vi "Initialize Hardware.vi"(7 "RT config file":path, 8 "error in":errorcluster, 11 "device parameters":T5) -> (0 "error out":errorcluster, 3 "RT handles":T4, 5 "device information":T1)   [LabVIEW 2020, in "Ballard ARINC 429 Engine.lvlib" / "Custom Device.lvlib"]
uses:
  Custom Device.lvlib
  Shared/Device Parameters.ctl
  Shared/Initialization Method.ctl
  Hardware Handles.ctl
  Device Information.ctl
  Hardware Direction and Channels.ctl
  Shared/Direction Capability.ctl
  <instrlib>/BTICardLib/Private/Initialize By Card Number and Core Number.vi
  <instrlib>/BTICardLib/Private/Initialize By Slot Number and Core Number.vi
  <instrlib>/BTICardLib/Private/Initialize By Core Serial Number.vi
  <instrlib>/BTICardLib/Private/IO/Action-Status/Write External LED.vi
  <instrlib>/BTI429Lib/Private/Core/Action-Status/Start All Channels.vi
  <instrlib>/BTICardLib/Private/Configure All From XML.vi
  <instrlib>/BTICardLib/BTICardLV.lvlib
  <instrlib>/BTI429Lib/BTI429LV.lvlib
  <vilib>/NI VeriStand/Custom Device Tools/Custom Device Utility Library/Custom Device Utility Library.lvlib
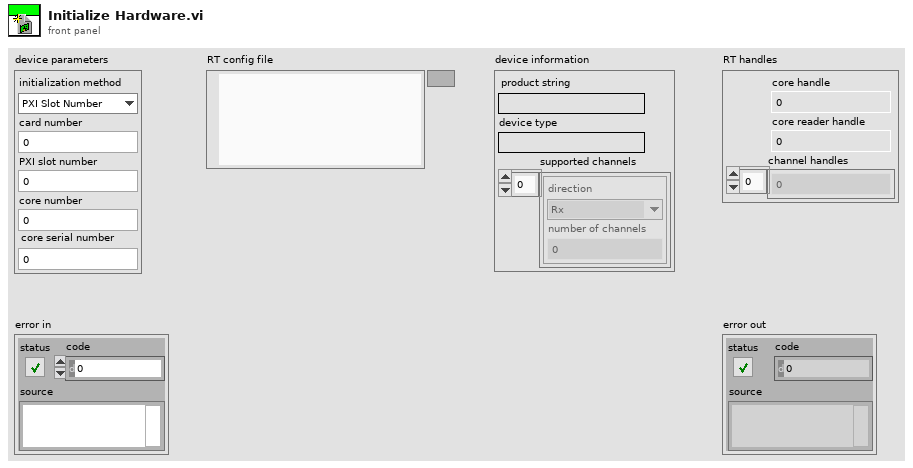
[diagram p1: front panel]
types:
  T1 = typedef "Ballard ARINC 429 Engine.lvlib/Custom Device.lvlib/Device Information.ctl" = cluster{"product string":string, "device type":string, "supported channels":T2[]}
  T2 = typedef "Ballard ARINC 429 Engine.lvlib/Custom Device.lvlib/Hardware Direction and Channels.ctl" = cluster{"direction":T3, "number of channels":u16}
  T3 = typedef "Direction Capability.ctl" = enum16{"Rx", "Tx", "Rx/Tx"}
  T4 = typedef "Ballard ARINC 429 Engine.lvlib/Custom Device.lvlib/Hardware Handles.ctl" = cluster{"core handle":u64, "core reader handle":u64, "channel handles":u64[]}
  T5 = typedef "Device Parameters.ctl" = cluster{"initialization method":T6, "card number":i32, "PXI slot number":i32, "core number":i32, "core serial number":i32}
  T6 = typedef "Initialization Method.ctl" = enum16{"PXI Slot Number", "Card Number", "Core Serial Number"}
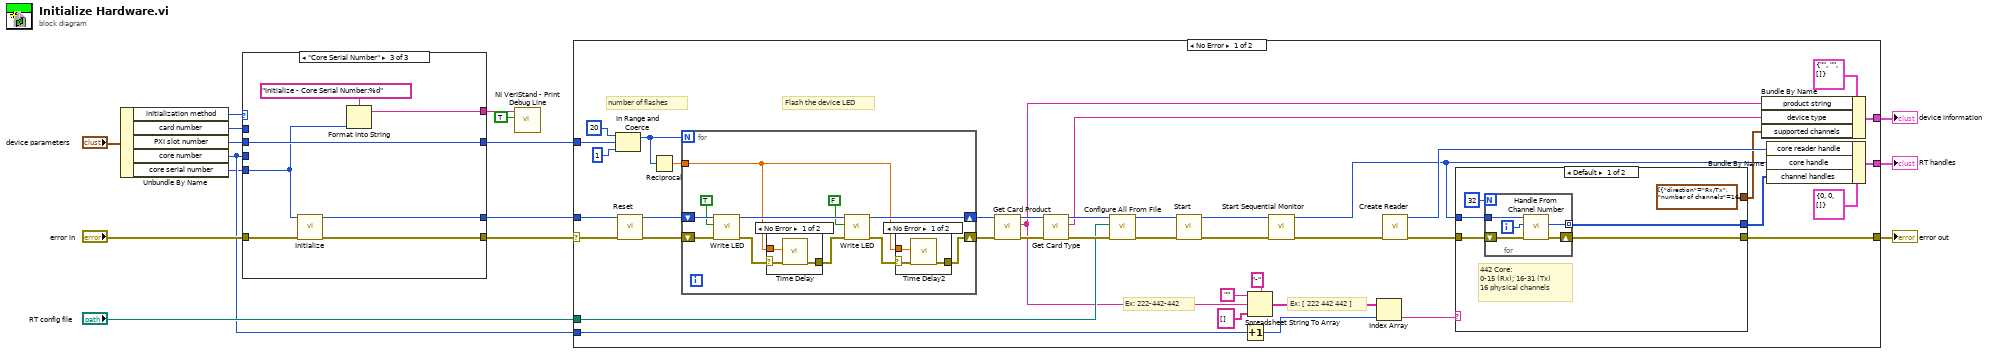
[diagram p0: block diagram]
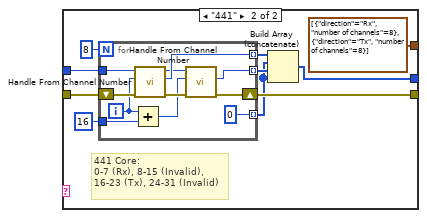
[diagram p2: hidden frame]
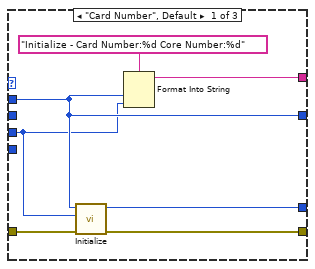
[diagram p6: hidden frame]
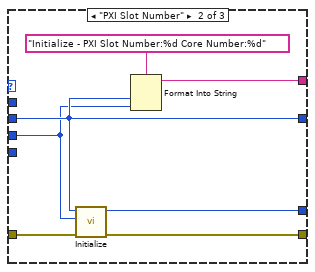
[diagram p7: hidden frame]
diagram:
  n1 = Unbundle By Name("device parameters") -> ("initialization method"=w16:T6, "card number"=w15:i32, "PXI slot number"=w14:i32, "core number"=w4:i32, "core serial number"=w3:i32)
  n2 = case shown="\"Core Serial Number\"" w16 {
    tunnel: [w23 w30 w37] -> w10
    tunnel: [w22 w29 w36] -> w12
    tunnel: w15 -> [w20 _ _]
    tunnel: "error in" -> [w21 w28 w35]
    tunnel: w14 -> [_ w27 w34]
    tunnel: w4 -> [w19 w26 _]
    tunnel: [w20 w27 w34] -> w9
    tunnel: w3 -> [_ _ w33]
    tunnel: [w17 w24 w31] -> w1
    frame "Card Number", Default {
      n3 = call-poly <instrlib>:"Initialize.vi"("error in (no error)"=w21, "core number"=w19, "card number"=w20) -> ("error out"=w22:errorcluster, "core handle out"=w23:u64)  [unwired: 7 in]
      n4 = Format Into String(format string="Initialize - Card Number:%d Core Number:%d", w20, w19) -> (resulting string=w17:string)  [unwired: 2 in, 1 out]
    }
    frame "PXI Slot Number" {
      n5 = call-poly <instrlib>:"Initialize.vi"("error in (no error)"=w28, "core number"=w26, "slot number"=w27) -> ("error out"=w29:errorcluster, "core handle out"=w30:u64)  [unwired: 7 in]
      n6 = Format Into String(format string="Initialize - PXI Slot Number:%d Core Number:%d", w27, w26) -> (resulting string=w24:string)  [unwired: 2 in, 1 out]
    }
    frame "Core Serial Number" {
      n7 = call-poly <instrlib>:"Initialize.vi"("error in (no error)"=w35, "core serial number"=w33) -> ("error out"=w36:errorcluster, "core handle out"=w37:u64)  [unwired: 8 in]
      n8 = Format Into String(format string="Initialize - Core Serial Number:%d", w33) -> (resulting string=w31:string)  [unwired: 2 in, 1 out]
    }
  }
  n9 = call <vilib>:"NI VeriStand - Print Debug Line.vi"("Add to log file? (F)"=TRUE, "Message"=w1) -> ()  [unwired: 9 in, 1 out]
  n10 = case shown="No Error" w12 {
    selector: w12 -> [w77 w128]
    tunnel: w10 -> [w76 _]
    tunnel: w9 -> [w73 _]
    tunnel: [w54 _] -> w8
    tunnel: [w52 _] -> w7
    tunnel: [w51 w128] -> w6
    tunnel: "RT config file" -> [w48 _]
    tunnel: w4 -> [w40 _]
    frame No Error {
      # "Ex: [ 222 442 442 ]"
      # "Ex: 222-442-442"
      # "number of flashes"
      # "Flash the device LED"
      n11 = In Range and Coerce(upper limit=20 ("x"), x=w73, lower limit=1) -> (coerced(x)=w69:i32)  [unwired: 1 out]
      n12 = call <instrlib>:"Reset.vi"("error in (no error)"=w77, "core handle in"=w76) -> ("error out"=w75:errorcluster, "core handle out"=w74:u64)  [unwired: 8 in]
      n13 = Reciprocal(x=w69) -> (1/x=w70:dbl)
      n14 = for {
        N: w69 -> [_]
        shift-right: [w118] -> w66
        shift-left: w74 -> [w117]
        shift-right: [w112] -> w65
        shift-left: w75 -> [w116]
        tunnel: w70 -> [w109]
        n15 = call-poly <instrlib>:"Write LED.vi"("error in (no error)"=w116, "LED state"=TRUE, "core handle in"=w117) -> ("error out"=w111:errorcluster, "core handle out"=w119:u64)  [unwired: 7 in]
        n16 = case shown="No Error" w111 {
          selector: w111 -> [w122 w123]
          tunnel: [w121 w123] -> w110
          tunnel: w109 -> [w120 _]
          frame No Error {
            n17 = call "Time Delay"("error in (no error)"=w122, "Delay Time (s)"=w120) -> ("error out"=w121:errorcluster)  [unwired: 9 in]
          }
          frame Error {
          }
        }
        n18 = call-poly <instrlib>:"Write LED.vi"("error in (no error)"=w110, "LED state"=FALSE, "core handle in"=w119) -> ("error out"=w113:errorcluster, "core handle out"=w118:u64)  [unwired: 7 in]
        n19 = case shown="No Error" w113 {
          selector: w113 -> [w126 w127]
          tunnel: [w125 w127] -> w112
          tunnel: w109 -> [w124 _]
          frame No Error {
            n20 = call "Time Delay2"("error in (no error)"=w126, "Delay Time (s)"=w124) -> ("error out"=w125:errorcluster)  [unwired: 9 in]
          }
          frame Error {
          }
        }
      }
      n21 = call <instrlib>:"Get Card Product.vi"("error in (no error)"=w65, "core handle in"=w66) -> ("error out"=w67:errorcluster, "product string out"=w42:string, "core handle out"=w68:u64)  [unwired: 7 in]
      n22 = call <instrlib>:"Get Card Type.vi"("error in (no error)"=w67, "core handle in"=w68) -> ("error out"=w57:errorcluster, "type string out"=w56:string, "core handle out"=w58:u64)  [unwired: 7 in]
      n23 = call-poly <instrlib>:"Configure All From File.vi"("error in (no error)"=w57, "configuration file path"=w48, "core handle in"=w58) -> ("error out"=w60:errorcluster, "core handle out"=w61:u64)  [unwired: 7 in]
      n24 = call-poly <instrlib>:"Start.vi"("error in (no error)"=w60, "core handle in"=w61) -> ("error out"=w63:errorcluster, "core handle out"=w62:u64)  [unwired: 8 in]
      n25 = Increment(x=w40) -> (x+1=w43:i32)
      n26 = Spreadsheet String To Array(delimiter (Tab)="-", format string="", spreadsheet string=w42, array type (2D Dbl)=string[] []) -> (array=w44:string[])
      n27 = call <instrlib>:"Start Sequential Monitor.vi"("error in (no error)"=w63, "core handle in"=w62) -> ("error out"=w64:errorcluster, "core handle out"=w47:u64)  [unwired: 8 in]
      n28 = Index Array(array=w44, index=w43) -> (element=w39:string)
      n29 = call <instrlib>:"Create Reader.vi"("error in (no error)"=w64) -> ("error out"=w59:errorcluster, "core reader handle out"=w49:u64)  [unwired: 9 in]
      n30 = case shown="Default" w39 {
        tunnel: w59 -> [w82 w97]
        tunnel: [w81 w96] -> w51
        tunnel: [w80 w90] -> w50
        tunnel: w47 -> [w79 w95]
        tunnel: [T2[] [{"direction"=enum."Rx/Tx", "number of channels"=16}] ("supported channels") T2[] [{"direction"=enum."Rx", "number of channels"=8}, {"direction"=enum."Tx", "number of channels"=8}] ("supported channels")] -> w38
        frame Default {
          # "442 Core:\n0-15 (Rx); 16-31 (Tx)\n16 physical channels"
          n31 = for {
            N: 32 -> [_]
            shift-right: [w85] -> w81
            shift-left: w82 -> [w88]
            tunnel: [w86] -> w80 mode=indexing
            tunnel: w79 -> [w84]
            i -> [w87]
            n32 = call <instrlib>:"Handle From Channel Number.vi"("error in (no error)"=w88, "channel number"=w87, "core handle in"=w84) -> ("error out"=w85:errorcluster, "channel handle out"=w86:u64)  [unwired: 6 in, 1 out]
          }
        }
        frame "441" {
          # "441 Core:\n0-7 (Rx), 8-15 (Invalid),\n16-23 (Tx), 24-31 (Invalid)"
          n33 = for {
            N: 8 -> [_]
            shift-right: [w106] -> w96
            shift-left: w97 -> [w108]
            tunnel: [w107] -> w94 mode=indexing
            tunnel: w95 -> [w105]
            tunnel: [w99] -> w93 mode=indexing
            tunnel: 16 ("y") -> [w101]
            tunnel: [u64 0 ("channel handle out")] -> w91 mode=indexing
            i -> [w103]
            n34 = Add(x=w103, y=w101) -> (x+y=w102:i32)
            n35 = call <instrlib>:"Handle From Channel Number.vi"("error in (no error)"=w108, "channel number"=w103, "core handle in"=w105) -> ("error out"=w106:errorcluster, "channel handle out"=w107:u64, "core handle out"=w104:u64)  [unwired: 6 in]
            n36 = call <instrlib>:"Handle From Channel Number.vi"("channel number"=w102, "core handle in"=w104) -> ("channel handle out"=w99:u64)  [unwired: 7 in, 2 out]
          }
          n37 = Build Array (concatenate)(w94, w91, w93, w91) -> (w90:u64[])
        }
      }
      n38 = Bundle By Name(cluster=T1 {"product string"="", "device type"="", "supported channels"=[]} ("hardware information"), "product string"=w42, "device type"=w56, "supported channels"=w38) -> (w54:T1)
      n39 = Bundle By Name(cluster=T4 {"core handle"=0, "core reader handle"=0, "channel handles"=[]} ("hardware handles"), "core reader handle"=w49, "core handle"=w47, "channel handles"=w50) -> (w52:T4)
    }
    frame Error {
    }
  }
  "RT handles" <- w7
  "error out" <- w6
  "device information" <- w8
